vi "Parse Auto Data.vi"(0 "path":path) -> (1 "Overall":cluster{"Time (s)":dbl, "Distance (ft)":dbl}, 3 "Commands out":cluster{"Time (s)":dbl, T1, bool}[](array[cluster]), 4 "Positions":cluster{"x":dbl, "y":dbl, "th":dbl}[](array[cluster]), 6 "Velocities":T3[](array[typedef]), 8 "Ball Pickup":bool, 10 "Zero Velocity?":bool[](array[boolean]), 13 "Correct at Beginning \nof Path":bool, 14 "Current Limit":dbl, 15 "Zero Translational Velocity?":bool[](array[boolean]))   [LabVIEW 2027]
uses:
  swerve-template/Type Definitions/Data/Robot Velocities.ctl
  bordeaux/Bordeaux/Types/Single Cmd Info.ctl
  <vilib>/picture/picture.llb/imagedata.ctl
  <vilib>/Analysis/coordinate.llb/2D Cartesian Coordinate Rotation (Scalar).vi
  <vilib>/Analysis/NI_AALPro.lvlib
  <vilib>/MRC/MrcLib.lvlib
panel:
  in  "Is Blue Alliance":bool=TRUE
  out "XY Graph":cluster{dbl[], dbl[]}[](graph)
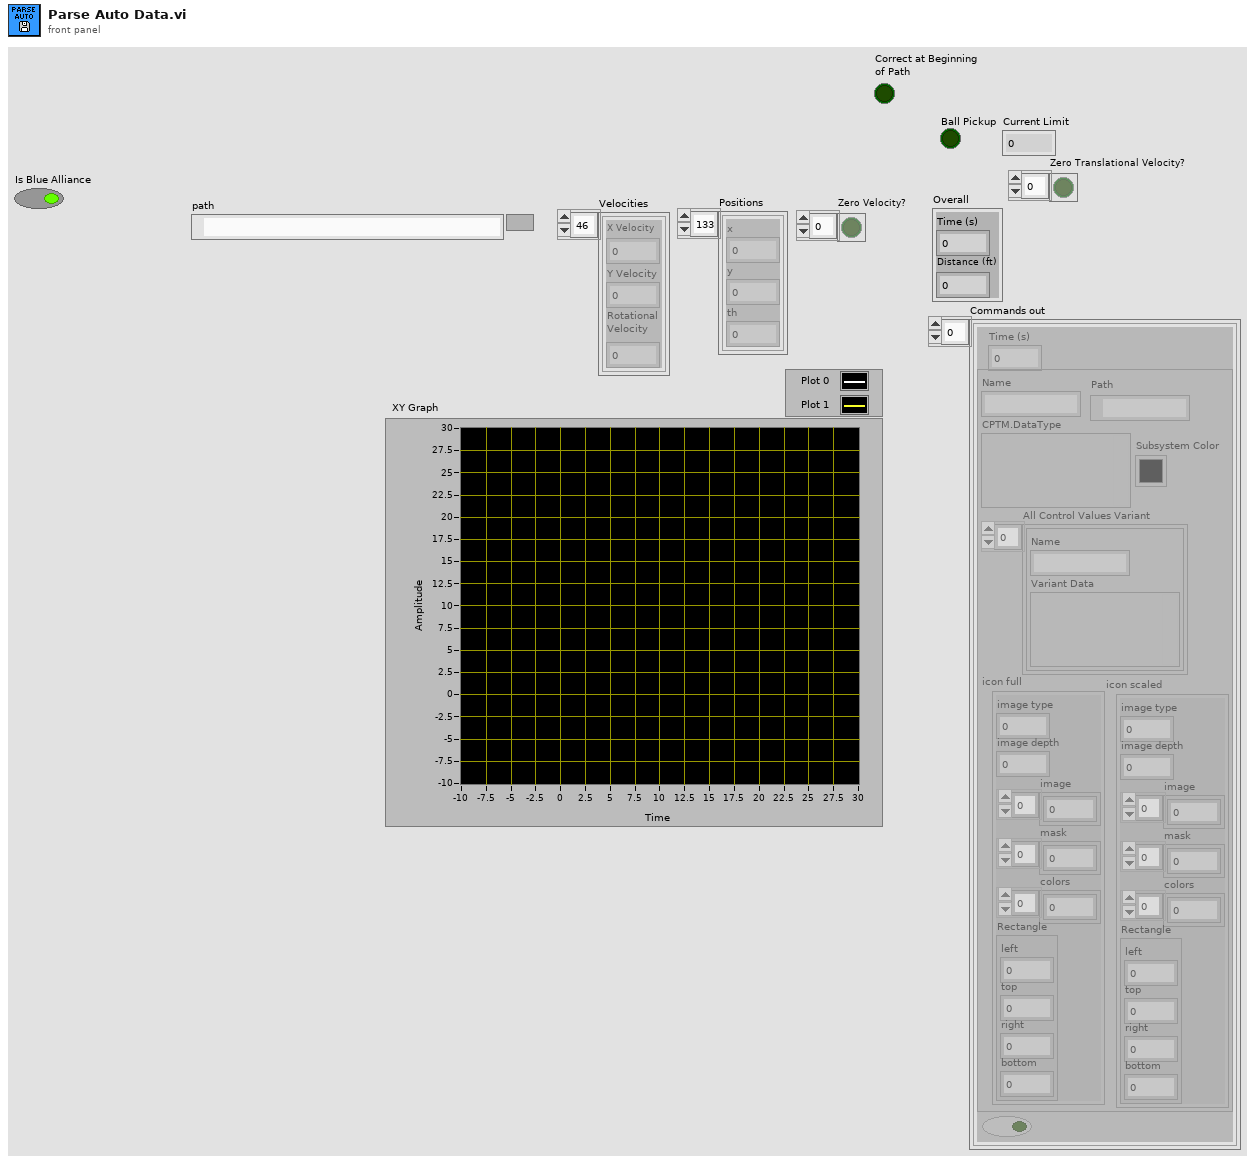
[diagram p1: front panel]
types:
  T1 = typedef "Single Cmd Info.ctl" = cluster{"Name":string, "CPTM.DataType":variant, "All Control Values Variant":cluster{"Name":string, "Variant Data":variant}[], "icon full":T2, "icon scaled":T2, "Path":path, "Subsystem Color":u32}
  T2 = typedef "imagedata.ctl" = cluster{"image type":i32, "image depth":i32, "image":u8[], "mask":u8[], "colors":u32[], "Rectangle":cluster{"left":i16, "top":i16, "right":i16, "bottom":i16}}
  T3 = typedef "Robot Velocities.ctl" = cluster{"X Velocity":dbl, "Y Velocity":dbl, "Rotational \nVelocity":dbl}
  T4 = typedef "WPI_DriverStationAllianceInfo.ctl" = enum16{"Red", "Blue", "Invalid"}
  T5 = typedef "WPI_DriverStationPositionInfo.ctl" = enum16{"1", "2", "3"}
  T6 = typedef "Trajectory Data.ctl" = cluster{"Segment Name":string, "Type":T7, "Traj Pos Points":cluster{"x":dbl, "y":dbl, "th":dbl}[], "Traj Vel Points":cluster{"V":dbl, "Omega":dbl, "V vector":cluster{"y":dbl, "x":dbl}}[], "Accel Index":i32, "Decel Index":i32}[]
  T7 = typedef "Segment Type.ctl" = enum16{"Accel Straight", "Const Straight", "Blend", "Circle", "Bezier"}
  T8 = cluster{"V":dbl, "Omega":dbl, "V vector":cluster{"y":dbl, "x":dbl}}[]
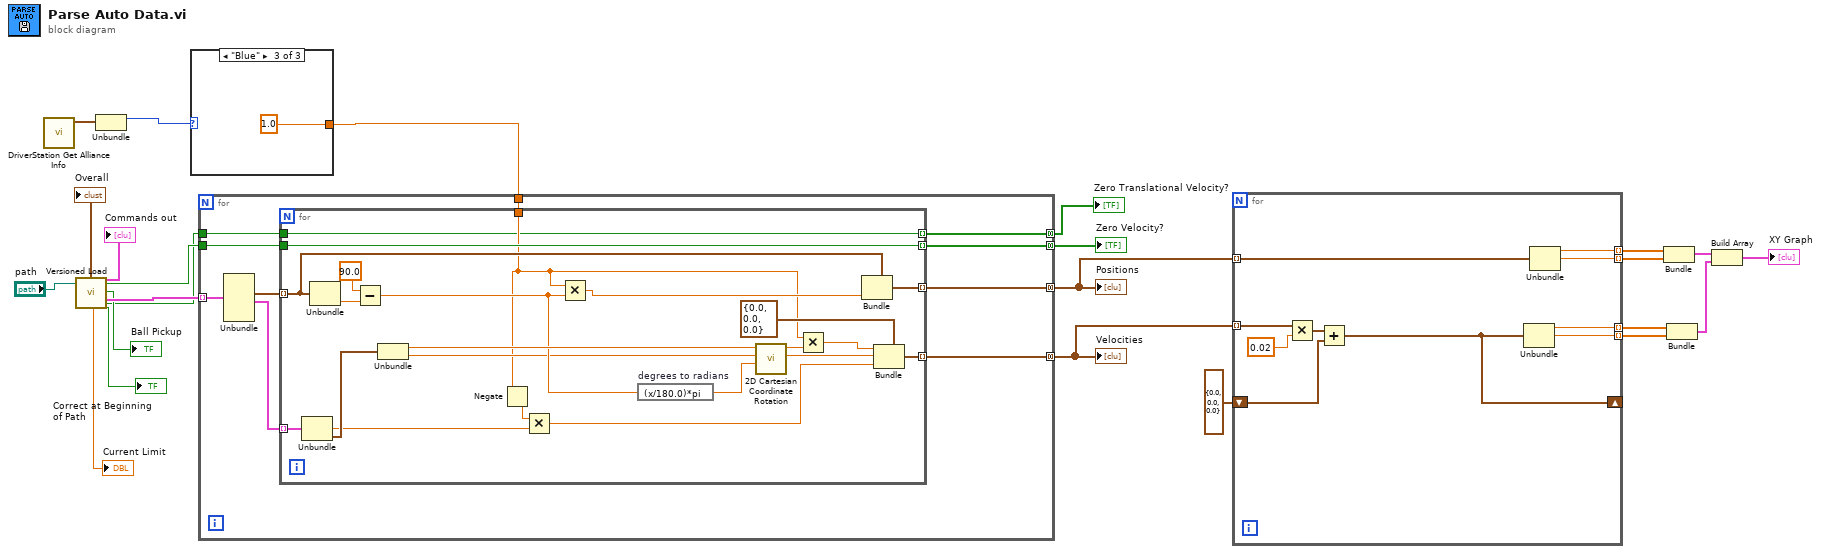
[diagram p0: block diagram]
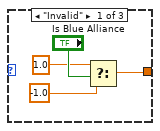
[diagram p2: hidden frame]
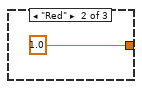
[diagram p3: hidden frame]
diagram:
  n1 = call <vilib>:"DriverStation Get Alliance Info.vi"() -> ("Alliance"=w2:cluster{"Color":T4, "Position":T5})  [unwired: 7 in, 4 out]
  n2 = call "Versioned Load.vi"("path"="path") -> ("Overall"=→"Overall":cluster{"Time (s)":dbl, "Distance (ft)":dbl}, "Current Limit"=→"Current Limit":dbl, "Commands out"=→"Commands out":cluster{"Time (s)":dbl, T1, bool}[], "Zero V"=w23:bool, "Ball Pickup"=→"Ball Pickup":bool, "Trajectory Data"=w24:T6, "Zero Translational Velocity"=w5:bool, "Correct at Beginning \nof Path"=→"Correct at Beginning \nof Path":bool)  [unwired: 15 in, 4 out]
  n3 = Unbundle(w2) -> ("Color"=w1:T4)  [unwired: 1 out]
  n4 = case shown="\"Blue\"" w1 {
    tunnel: [w25 1.0 1.0] -> w9
    frame "Invalid" {
      n5 = Select(t=1.0, s="Is Blue Alliance", f=-1.0) -> (s? t:f=w25:dbl)
    }
    frame "Red" {
    }
    frame "Blue" {
    }
  }
  n6 = for {
    tunnel: w24 -> [w40] mode=indexing
    tunnel: [w37] -> w20 mode=concatenating
    tunnel: w9 -> [w36]
    tunnel: [w33] -> w19 mode=concatenating
    tunnel: w23 -> [w35]
    tunnel: [w34] -> w22 mode=concatenating
    tunnel: w5 -> [w32]
    tunnel: [w31] -> w4 mode=concatenating
    n7 = Unbundle(w40) -> ("Traj Pos Points"=w39:cluster{"x":dbl, "y":dbl, "th":dbl}[], "Traj Vel Points"=w38:T8)  [unwired: 4 out]
    n8 = for {
      tunnel: w39 -> [w60] mode=indexing
      tunnel: w38 -> [w58] mode=indexing
      tunnel: [w59] -> w37 mode=indexing
      tunnel: w36 -> [w42]
      tunnel: [w51] -> w33 mode=indexing
      tunnel: w35 -> [w48]
      tunnel: [w48] -> w34 mode=indexing
      tunnel: w32 -> [w41]
      tunnel: [w41] -> w31 mode=indexing
      n9 = Unbundle(w58) -> ("Omega"=w45:dbl, "V vector"=w57:cluster{"y":dbl, "x":dbl})  [unwired: 1 out]
      n10 = Unbundle(w60) -> ("th"=w62:dbl)  [unwired: 2 out]
      n11 = Subtract(x=90.0, y=w62) -> (x-y=w47:dbl)
      n12 = Unbundle(w57) -> ("y"=w55:dbl, "x"=w44:dbl)
      n13 = Negate(x=w42) -> (-x=w43:dbl)
      n14 = Multiply(x=w43, y=w45) -> (x*y=w53:dbl)
      n15 = Multiply(x=w42, y=w47) -> (x*y=w46:dbl)
      n16 = expression code="(x/180.0)*pi" "degrees to radians"(w47) -> (w56:dbl)
      n17 = call-poly <vilib>:"2D Cartesian Coordinate Rotation.vi"("theta"=w56, "y"=w44, "x"=w55) -> ("y out"=w54:dbl, "x out"=w50:dbl)  [unwired: 6 in, 1 out]
      n18 = Multiply(x=w42, y=w50) -> (x*y=w49:dbl)
      n19 = Bundle(cluster=w60, "th"=w46) -> (w59:cluster{"x":dbl, "y":dbl, "th":dbl})  [unwired: 2 in]
      n20 = Bundle(cluster=T3 {"X Velocity"=0.0, "Y Velocity"=0.0, "Rotational \nVelocity"=0.0} ("Robot Velocities"), "X Velocity"=w49, "Y Velocity"=w54, "Rotational \nVelocity"=w53) -> (w51:T3)
    }
  }
  "Positions" <- w20
  "Velocities" <- w19
  "Zero Velocity?" <- w22
  "Zero Translational Velocity?" <- w4
  n21 = for {
    tunnel: w20 -> [w72] mode=indexing
    tunnel: w19 -> [w69] mode=indexing
    tunnel: [w71] -> w18 mode=indexing
    tunnel: [w70] -> w17 mode=indexing
    shift-right: [w65] -> _
    shift-left: T3 {"X Velocity"=0.0, "Y Velocity"=0.0, "Rotational \nVelocity"=0.0} ("Robot Velocities") -> [w66]
    tunnel: [w64] -> w16 mode=indexing
    tunnel: [w63] -> w15 mode=indexing
    n22 = Multiply(x=w69, y=0.02) -> (x*y=w67:T3)
    n23 = Add(x=w67, y=w66) -> (x+y=w65:T3)
    n24 = Unbundle(w65) -> ("X Velocity"=w64:dbl, "Y Velocity"=w63:dbl)  [unwired: 1 out]
    n25 = Unbundle(w72) -> ("x"=w71:dbl, "y"=w70:dbl)  [unwired: 1 out]
  }
  n26 = Bundle(w18, w17) -> (w14:cluster{dbl[], dbl[]})  [unwired: 1 in]
  n27 = Bundle(w16, w15) -> (w13:cluster{dbl[], dbl[]})  [unwired: 1 in]
  n28 = Build Array(w14, w13) -> (→"XY Graph":cluster{dbl[], dbl[]}[])
